vi "IV_.vi"(9 "B rate":dbl=0.02, 10 "Notes":string="LAOSTO110_2.K.20140812\n\nVbg=0.3V\nsweep Bx: 0T --> 1T --> -1T --> 0T, 0.02T/min\n\nLockin\n0:2\n1: 20\n2: 21\n3: 22\n4: 23\n5: 24\n\n", 11 "Experiment folder name":string="1 - sweep B,IV") -> ()   [LabVIEW 2013]
uses:
  <vilib>/Analysis/2dsp.llb/Decimate (single shot, DBL).vi
  <userlib>/LevyLab/PPMS VI/SubVI/ITX_Global.vi
  P:/users1/Joe/Lockin-4461_3.0 4461-4462 Multichannel Folder/DAQ-Lockin-SubVI/Lock-in Globles Multiple Inputs and Outputs.vi
  Q:/inst/Leiden measurements VIs/IV measurement/Sub VIs/Global Value.vi
  B field global.vi
  <vilib>/Analysis/NI_AALPro.lvlib
panel:
  out "4Term 2":cluster{dbl[], dbl[]}[](graph)
  out "4Term":cluster{dbl[], dbl[]}[](graph)
  out "2Term":cluster{dbl[], dbl[]}[](graph)
  in  "Tab Control":enum32{"Settings", "ITX", "Lockin Data"}(tab)
  in  "Current Channel 1":i32
  in  "Source Channel":i32
  in  "decimating factor":i32=400
  in  "low cutoff freq: fl":dbl=0.03 format="%0.4f"
  out "Gains":dbl[](array[numeric])=[50000000.0, 1000.0, 1000.0, 1000.0, 50000000.0, 1000.0]
  out "time":dbl[](array[numeric])=[3490742841.6947465, 3490742841.6967463, 3490742841.6987467, 3490742841.7007465, 3490742841.7027464, 3490742841.7047467, 3490742841.7067466, 3490742841.7087464, 3490742841.7107463, 3490742841.7127466, 3490742841.7147465, 3490742841.7167463, 3490742841.7187467, 3490742841.7207465, 3490742841.7227464, 3490742841.7247467, 3490742841.7267466, 3490742841.7287464, 3490742841.7307463, 3490742841.7327466, 3490742841.7347465, 3490742841.7367463, 3490742841.7387466, 3490742841.7407465, 3490742841.7427464, 3490742841.7447467, 3490742841.7467465, 3490742841.7487464, 3490742841.7507467, 3490742841.7527466, 3490742841.7547464, 3490742841.7567463, 3490742841.7587466, 3490742841.7607465, 3490742841.7627463, 3490742841.7647467, 3490742841.7667465, 3490742841.7687464, 3490742841.7707467, 3490742841.7727466, 3490742841.7747464, 3490742841.7767463, 3490742841.7787466, 3490742841.7807465, 3490742841.7827463, 3490742841.7847466, 3490742841.7867465, 3490742841.7887464, 3490742841.7907467, 3490742841.7927465, 3490742841.7947464, 3490742841.7967467, 3490742841.7987466, 3490742841.8007464, 3490742841.8027463, 3490742841.8047466, 3490742841.8067465, 3490742841.8087463, 3490742841.8107467, 3490742841.8127465, 3490742841.8147464, 3490742841.8167467, 3490742841.8187466, 3490742841.8207464, 3490742841.8227463, 3490742841.8247466, 3490742841.8267465, 3490742841.8287463, 3490742841.8307467, 3490742841.8327465, 3490742841.8347464, 3490742841.8367467, 3490742841.8387465, 3490742841.8407464, 3490742841.8427463, 3490742841.8447466, 3490742841.8467464, 3490742841.8487463, 3490742841.8507466, 3490742841.8527465, 3490742841.8547463, 3490742841.8567467, 3490742841.8587465, 3490742841.8607464, 3490742841.8627467, 3490742841.8647466, 3490742841.8667464, 3490742841.8687463, 3490742841.8707466, 3490742841.8727465, 3490742841.8747463, 3490742841.8767467, 3490742841.8787465, 3490742841.8807464, 3490742841.8827467, 3490742841.8847466, 3490742841.8867464, 3490742841.8887463, 3490742841.8907466, 3490742841.8927464, 3490742841.8947463, 3490742841.8967466, 3490742841.8987465, 3490742841.9007463, 3490742841.9027467, 3490742841.9047465, 3490742841.9067464, 3490742841.9087467, 3490742841.9107466, 3490742841.9127464, 3490742841.9147463, 3490742841.9167466, 3490742841.9187465, 3490742841.9207463, 3490742841.9227467, 3490742841.9247465, 3490742841.9267464, 3490742841.9287467, 3490742841.9307466, 3490742841.9327464, 3490742841.9347463, 3490742841.9367466, 3490742841.9387465, 3490742841.9407463, 3490742841.9427466, 3490742841.9447465, 3490742841.9467463, 3490742841.9487467, 3490742841.9507465, 3490742841.9527464, 3490742841.9547467, 3490742841.9567466, 3490742841.9587464, 3490742841.9607463, 3490742841.9627466, 3490742841.9647465, 3490742841.9667463, 3490742841.9687467, 3490742841.9707465, 3490742841.9727464, 3490742841.9747467, 3490742841.9767466, 3490742841.9787464, 3490742841.9807463, 3490742841.9827466, 3490742841.9847465, 3490742841.9867463, 3490742841.9887466, 3490742841.9907465, 3490742841.9927464, 3490742841.9947467, 3490742841.9967465, 3490742841.9987464, 3490742842.0007467, 3490742842.0027466, 3490742842.0047464, 3490742842.0067463, 3490742842.0087466, 3490742842.0107465, 3490742842.0127463, 3490742842.0147467, 3490742842.0167465, 3490742842.0187464, 3490742842.0207467, 3490742842.0227466, 3490742842.0247464, 3490742842.0267463, 3490742842.0287466, 3490742842.0307465, 3490742842.0327463, 3490742842.0347466, 3490742842.0367465, 3490742842.0387464, 3490742842.0407467, 3490742842.0427465, 3490742842.0447464, 3490742842.0467467, 3490742842.0487466, 3490742842.0507464, 3490742842.0527463, 3490742842.0547466, 3490742842.0567465, 3490742842.0587463, 3490742842.0607467, 3490742842.0627465, 3490742842.0647464, 3490742842.0667467, 3490742842.0687466, 3490742842.0707464, 3490742842.0727463, 3490742842.0747466, 3490742842.0767465, 3490742842.0787463, 3490742842.0807467, 3490742842.0827465, 3490742842.0847464, 3490742842.0867467, 3490742842.0887465, 3490742842.0907464, 3490742842.0927463, 3490742842.0947466, 3490742842.0967464, 3490742842.0987463, 3490742842.1007466, 3490742842.1027465, 3490742842.1047463, 3490742842.1067467, 3490742842.1087465, 3490742842.1107464, 3490742842.1127467, 3490742842.1147466, 3490742842.1167464, 3490742842.1187463, 3490742842.1207466, 3490742842.1227465, 3490742842.1247463, 3490742842.1267467, 3490742842.1287465, 3490742842.1307464, 3490742842.1327467, 3490742842.1347466, 3490742842.1367464, 3490742842.1387463, 3490742842.1407466, 3490742842.1427464, 3490742842.1447463, 3490742842.1467466, 3490742842.1487465, 3490742842.1507463, 3490742842.1527467, 3490742842.1547465, 3490742842.1567464, 3490742842.1587467, 3490742842.1607466, 3490742842.1627464, 3490742842.1647463, 3490742842.1667466, 3490742842.1687465, 3490742842.1707463, 3490742842.1727467, 3490742842.1747465, 3490742842.1767464, 3490742842.1787467, 3490742842.1807466, 3490742842.1827464, 3490742842.1847463, 3490742842.1867466, 3490742842.1887465, 3490742842.1907463, 3490742842.1927466, 3490742842.1947465, 3490742842.1967463, 3490742842.1987467, 3490742842.2007465, 3490742842.2027464, 3490742842.2047467, 3490742842.2067466, 3490742842.2087464, 3490742842.2107463, 3490742842.2127466, 3490742842.2147465, 3490742842.2167463, 3490742842.2187467, 3490742842.2207465, 3490742842.2227464, 3490742842.2247467, 3490742842.2267466, 3490742842.2287464, 3490742842.2307463, 3490742842.2327466, 3490742842.2347465, 3490742842.2367463, 3490742842.2387466, 3490742842.2407465, 3490742842.2427464, 3490742842.2447467, 3490742842.2467465, 3490742842.2487464, 3490742842.2507467, 3490742842.2527466, 3490742842.2547464, 3490742842.2567463, 3490742842.2587466, 3490742842.2607465, 3490742842.2627463, 3490742842.2647467, 3490742842.2667465, 3490742842.2687464, 3490742842.2707467, 3490742842.2727466, 3490742842.2747464, 3490742842.2767463, 3490742842.2787466, 3490742842.2807465, 3490742842.2827463, 3490742842.2847466, 3490742842.2867465, 3490742842.2887464, 3490742842.2907467, 3490742842.2927465, 3490742842.2947464, 3490742842.2967467, 3490742842.2987466, 3490742842.3007464, 3490742842.3027463, 3490742842.3047466, 3490742842.3067465, 3490742842.3087463, 3490742842.3107467, 3490742842.3127465, 3490742842.3147464, 3490742842.3167467, 3490742842.3187466, 3490742842.3207464, 3490742842.3227463, 3490742842.3247466, 3490742842.3267465, 3490742842.3287463, 3490742842.3307467, 3490742842.3327465, 3490742842.3347464, 3490742842.3367467, 3490742842.3387465, 3490742842.3407464, 3490742842.3427463, 3490742842.3447466, 3490742842.3467464, 3490742842.3487463, 3490742842.3507466, 3490742842.3527465, 3490742842.3547463, 3490742842.3567467, 3490742842.3587465, 3490742842.3607464, 3490742842.3627467, 3490742842.3647466, 3490742842.3667464, 3490742842.3687463, 3490742842.3707466, 3490742842.3727465, 3490742842.3747463, 3490742842.3767467, 3490742842.3787465, 3490742842.3807464, 3490742842.3827467, 3490742842.3847466, 3490742842.3867464, 3490742842.3887463, 3490742842.3907466, 3490742842.3927464, 3490742842.3947463, 3490742842.3967466, 3490742842.3987465, 3490742842.4007463, 3490742842.4027467, 3490742842.4047465, 3490742842.4067464, 3490742842.4087467, 3490742842.4107466, 3490742842.4127464, 3490742842.4147463, 3490742842.4167466, 3490742842.4187465, 3490742842.4207463, 3490742842.4227467, 3490742842.4247465, 3490742842.4267464, 3490742842.4287467, 3490742842.4307466, 3490742842.4327464, 3490742842.4347463, 3490742842.4367466, 3490742842.4387465, 3490742842.4407463, 3490742842.4427466, 3490742842.4447465, 3490742842.4467463, 3490742842.4487467, 3490742842.4507465, 3490742842.4527464, 3490742842.4547467, 3490742842.4567466, 3490742842.4587464, 3490742842.4607463, 3490742842.4627466, 3490742842.4647465, 3490742842.4667463, 3490742842.4687467, 3490742842.4707465, 3490742842.4727464, 3490742842.4747467, 3490742842.4767466, 3490742842.4787464, 3490742842.4807463, 3490742842.4827466, 3490742842.4847465, 3490742842.4867463, 3490742842.4887466, 3490742842.4907465, 3490742842.4927464, 3490742842.4947467, 3490742842.4967465, 3490742842.4987464, 3490742842.5007467, 3490742842.5027466, 3490742842.5047464, 3490742842.5067463, 3490742842.5087466, 3490742842.5107465, 3490742842.5127463, 3490742842.5147467, 3490742842.5167465, 3490742842.5187464, 3490742842.5207467, 3490742842.5227466, 3490742842.5247464, 3490742842.5267463, 3490742842.5287466, 3490742842.5307465, 3490742842.5327463, 3490742842.5347466, 3490742842.5367465, 3490742842.5387464, 3490742842.5407467, 3490742842.5427465, 3490742842.5447464, 3490742842.5467467, 3490742842.5487466, 3490742842.5507464, 3490742842.5527463, 3490742842.5547466, 3490742842.5567465, 3490742842.5587463, 3490742842.5607467, 3490742842.5627465, 3490742842.5647464, 3490742842.5667467, 3490742842.5687466, 3490742842.5707464, 3490742842.5727463, 3490742842.5747466, 3490742842.5767465, 3490742842.5787463, 3490742842.5807467, 3490742842.5827465, 3490742842.5847464, 3490742842.5867467, 3490742842.5887465, 3490742842.5907464, 3490742842.5927463, 3490742842.5947466, 3490742842.5967464, 3490742842.5987463, 3490742842.6007466, 3490742842.6027465, 3490742842.6047463, 3490742842.6067467, 3490742842.6087465, 3490742842.6107464, 3490742842.6127467, 3490742842.6147466, 3490742842.6167464, 3490742842.6187463, 3490742842.6207466, 3490742842.6227465, 3490742842.6247463, 3490742842.6267467, 3490742842.6287465, 3490742842.6307464, 3490742842.6327467, 3490742842.6347466, 3490742842.6367464, 3490742842.6387463, 3490742842.6407466, 3490742842.6427464, 3490742842.6447463, 3490742842.6467466, 3490742842.6487465, 3490742842.6507463, 3490742842.6527467, 3490742842.6547465, 3490742842.6567464, 3490742842.6587467, 3490742842.6607466, 3490742842.6627464, 3490742842.6647463, 3490742842.6667466, 3490742842.6687465, 3490742842.6707463, 3490742842.6727467, 3490742842.6747465, 3490742842.6767464, 3490742842.6787467, 3490742842.6807466, 3490742842.6827464, 3490742842.6847463, 3490742842.6867466, 3490742842.6887465, 3490742842.6907463, 3490742842.6927466, 3490742842.6947465, 3490742842.6967463, 3490742842.6987467, 3490742842.7007465, 3490742842.7027464, 3490742842.7047467, 3490742842.7067466, 3490742842.7087464, 3490742842.7107463, 3490742842.7127466, 3490742842.7147465, 3490742842.7167463, 3490742842.7187467, 3490742842.7207465, 3490742842.7227464, 3490742842.7247467, 3490742842.7267466, 3490742842.7287464, 3490742842.7307463, 3490742842.7327466, 3490742842.7347465, 3490742842.7367463, 3490742842.7387466, 3490742842.7407465, 3490742842.7427464, 3490742842.7447467, 3490742842.7467465, 3490742842.7487464, 3490742842.7507467, 3490742842.7527466, 3490742842.7547464, 3490742842.7567463, 3490742842.7587466, 3490742842.7607465, 3490742842.7627463, 3490742842.7647467, 3490742842.7667465, 3490742842.7687464, 3490742842.7707467, 3490742842.7727466, 3490742842.7747464, 3490742842.7767463, 3490742842.7787466, 3490742842.7807465, 3490742842.7827463, 3490742842.7847466, 3490742842.7867465, 3490742842.7887464, 3490742842.7907467, 3490742842.7927465, 3490742842.7947464, 3490742842.7967467, 3490742842.7987466, 3490742842.8007464, 3490742842.8027463, 3490742842.8047466, 3490742842.8067465, 3490742842.8087463, 3490742842.8107467, 3490742842.8127465, 3490742842.8147464, 3490742842.8167467, 3490742842.8187466, 3490742842.8207464, 3490742842.8227463, 3490742842.8247466, 3490742842.8267465, 3490742842.8287463, 3490742842.8307467, 3490742842.8327465, 3490742842.8347464, 3490742842.8367467, 3490742842.8387465, 3490742842.8407464, 3490742842.8427463, 3490742842.8447466, 3490742842.8467464, 3490742842.8487463, 3490742842.8507466, 3490742842.8527465, 3490742842.8547463, 3490742842.8567467, 3490742842.8587465, 3490742842.8607464, 3490742842.8627467, 3490742842.8647466, 3490742842.8667464, 3490742842.8687463, 3490742842.8707466, 3490742842.8727465, 3490742842.8747463, 3490742842.8767467, 3490742842.8787465, 3490742842.8807464, 3490742842.8827467, 3490742842.8847466, 3490742842.8867464, 3490742842.8887463, 3490742842.8907466, 3490742842.8927464, 3490742842.8947463, 3490742842.8967466, 3490742842.8987465, 3490742842.9007463, 3490742842.9027467, 3490742842.9047465, 3490742842.9067464, 3490742842.9087467, 3490742842.9107466, 3490742842.9127464, 3490742842.9147463, 3490742842.9167466, 3490742842.9187465, 3490742842.9207463, 3490742842.9227467, 3490742842.9247465, 3490742842.9267464, 3490742842.9287467, 3490742842.9307466, 3490742842.9327464, 3490742842.9347463, 3490742842.9367466, 3490742842.9387465, 3490742842.9407463, 3490742842.9427466, 3490742842.9447465, 3490742842.9467463, 3490742842.9487467, 3490742842.9507465, 3490742842.9527464, 3490742842.9547467, 3490742842.9567466, 3490742842.9587464, 3490742842.9607463, 3490742842.9627466, 3490742842.9647465, 3490742842.9667463, 3490742842.9687467, 3490742842.9707465, 3490742842.9727464, 3490742842.9747467, 3490742842.9767466, 3490742842.9787464, 3490742842.9807463, 3490742842.9827466, 3490742842.9847465, 3490742842.9867463, 3490742842.9887466, 3490742842.9907465, 3490742842.9927464, 3490742842.9947467, 3490742842.9967465, 3490742842.9987464, 3490742843.0007467, 3490742843.0027466, 3490742843.0047464, 3490742843.0067463, 3490742843.0087466, 3490742843.0107465, 3490742843.0127463, 3490742843.0147467, 3490742843.0167465, 3490742843.0187464, 3490742843.0207467, 3490742843.0227466, 3490742843.0247464, 3490742843.0267463, 3490742843.0287466, 3490742843.0307465, 3490742843.0327463, 3490742843.0347466, 3490742843.0367465, 3490742843.0387464, 3490742843.0407467, 3490742843.0427465, 3490742843.0447464, 3490742843.0467467, 3490742843.0487466, 3490742843.0507464, 3490742843.0527463, 3490742843.0547466, 3490742843.0567465, 3490742843.0587463, 3490742843.0607467, 3490742843.0627465, 3490742843.0647464, 3490742843.0667467, 3490742843.0687466, 3490742843.0707464, 3490742843.0727463, 3490742843.0747466, 3490742843.0767465, 3490742843.0787463, 3490742843.0807467, 3490742843.0827465, 3490742843.0847464, 3490742843.0867467, 3490742843.0887465, 3490742843.0907464, 3490742843.0927463, 3490742843.0947466, 3490742843.0967464, 3490742843.0987463, 3490742843.1007466, 3490742843.1027465, 3490742843.1047463, 3490742843.1067467, 3490742843.1087465, 3490742843.1107464, 3490742843.1127467, 3490742843.1147466, 3490742843.1167464, 3490742843.1187463, 3490742843.1207466, 3490742843.1227465, 3490742843.1247463, 3490742843.1267467, 3490742843.1287465, 3490742843.1307464, 3490742843.1327467, 3490742843.1347466, 3490742843.1367464, 3490742843.1387463, 3490742843.1407466, 3490742843.1427464, 3490742843.1447463, 3490742843.1467466, 3490742843.1487465, 3490742843.1507463, 3490742843.1527467, 3490742843.1547465, 3490742843.1567464, 3490742843.1587467, 3490742843.1607466, 3490742843.1627464, 3490742843.1647463, 3490742843.1667466, 3490742843.1687465, 3490742843.1707463, 3490742843.1727467, 3490742843.1747465, 3490742843.1767464, 3490742843.1787467, 3490742843.1807466, 3490742843.1827464, 3490742843.1847463, 3490742843.1867466, 3490742843.1887465, 3490742843.1907463, 3490742843.1927466, 3490742843.1947465, 3490742843.1967463, 3490742843.1987467, 3490742843.2007465, 3490742843.2027464, 3490742843.2047467, 3490742843.2067466, 3490742843.2087464, 3490742843.2107463, 3490742843.2127466, 3490742843.2147465, 3490742843.2167463, 3490742843.2187467, 3490742843.2207465, 3490742843.2227464, 3490742843.2247467, 3490742843.2267466, 3490742843.2287464, 3490742843.2307463, 3490742843.2327466, 3490742843.2347465, 3490742843.2367463, 3490742843.2387466, 3490742843.2407465, 3490742843.2427464, 3490742843.2447467, 3490742843.2467465, 3490742843.2487464, 3490742843.2507467, 3490742843.2527466, 3490742843.2547464, 3490742843.2567463, 3490742843.2587466, 3490742843.2607465, 3490742843.2627463, 3490742843.2647467, 3490742843.2667465, 3490742843.2687464, 3490742843.2707467, 3490742843.2727466, 3490742843.2747464, 3490742843.2767463, 3490742843.2787466, 3490742843.2807465, 3490742843.2827463, 3490742843.2847466, 3490742843.2867465, 3490742843.2887464, 3490742843.2907467, 3490742843.2927465, 3490742843.2947464, 3490742843.2967467, 3490742843.2987466, 3490742843.3007464, 3490742843.3027463, 3490742843.3047466, 3490742843.3067465, 3490742843.3087463, 3490742843.3107467, 3490742843.3127465, 3490742843.3147464, 3490742843.3167467, 3490742843.3187466, 3490742843.3207464, 3490742843.3227463, 3490742843.3247466, 3490742843.3267465, 3490742843.3287463, 3490742843.3307467, 3490742843.3327465, 3490742843.3347464, 3490742843.3367467, 3490742843.3387465, 3490742843.3407464, 3490742843.3427463, 3490742843.3447466, 3490742843.3467464, 3490742843.3487463, 3490742843.3507466, 3490742843.3527465, 3490742843.3547463, 3490742843.3567467, 3490742843.3587465, 3490742843.3607464, 3490742843.3627467, 3490742843.3647466, 3490742843.3667464, 3490742843.3687463, 3490742843.3707466, 3490742843.3727465, 3490742843.3747463, 3490742843.3767467, 3490742843.3787465, 3490742843.3807464, 3490742843.3827467, 3490742843.3847466, 3490742843.3867464, 3490742843.3887463, 3490742843.3907466, 3490742843.3927464, 3490742843.3947463, 3490742843.3967466, 3490742843.3987465, 3490742843.4007463, 3490742843.4027467, 3490742843.4047465, 3490742843.4067464, 3490742843.4087467, 3490742843.4107466, 3490742843.4127464, 3490742843.4147463, 3490742843.4167466, 3490742843.4187465, 3490742843.4207463, 3490742843.4227467, 3490742843.4247465, 3490742843.4267464, 3490742843.4287467, 3490742843.4307466, 3490742843.4327464, 3490742843.4347463, 3490742843.4367466, 3490742843.4387465, 3490742843.4407463, 3490742843.4427466, 3490742843.4447465, 3490742843.4467463, 3490742843.4487467, 3490742843.4507465, 3490742843.4527464, 3490742843.4547467, 3490742843.4567466, 3490742843.4587464, 3490742843.4607463, 3490742843.4627466, 3490742843.4647465, 3490742843.4667463, 3490742843.4687467, 3490742843.4707465, 3490742843.4727464, 3490742843.4747467, 3490742843.4767466, 3490742843.4787464, 3490742843.4807463, 3490742843.4827466, 3490742843.4847465, 3490742843.4867463, 3490742843.4887466, 3490742843.4907465, 3490742843.4927464, 3490742843.4947467, 3490742843.4967465, 3490742843.4987464, 3490742843.5007467, 3490742843.5027466, 3490742843.5047464, 3490742843.5067463, 3490742843.5087466, 3490742843.5107465, 3490742843.5127463, 3490742843.5147467, 3490742843.5167465, 3490742843.5187464, 3490742843.5207467, 3490742843.5227466, 3490742843.5247464, 3490742843.5267463, 3490742843.5287466, 3490742843.5307465, 3490742843.5327463, 3490742843.5347466, 3490742843.5367465, 3490742843.5387464, 3490742843.5407467, 3490742843.5427465, 3490742843.5447464, 3490742843.5467467, 3490742843.5487466, 3490742843.5507464, 3490742843.5527463, 3490742843.5547466, 3490742843.5567465, 3490742843.5587463, 3490742843.5607467, 3490742843.5627465, 3490742843.5647464, 3490742843.5667467, 3490742843.5687466, 3490742843.5707464, 3490742843.5727463, 3490742843.5747466, 3490742843.5767465, 3490742843.5787463, 3490742843.5807467, 3490742843.5827465, 3490742843.5847464, 3490742843.5867467, 3490742843.5887465, 3490742843.5907464, 3490742843.5927463, 3490742843.5947466, 3490742843.5967464, 3490742843.5987463, 3490742843.6007466, 3490742843.6027465, 3490742843.6047463, 3490742843.6067467, 3490742843.6087465, 3490742843.6107464, 3490742843.6127467, 3490742843.6147466, 3490742843.6167464, 3490742843.6187463, 3490742843.6207466, 3490742843.6227465, 3490742843.6247463, 3490742843.6267467, 3490742843.6287465, 3490742843.6307464, 3490742843.6327467, 3490742843.6347466, 3490742843.6367464, 3490742843.6387463, 3490742843.6407466, 3490742843.6427464, 3490742843.6447463, 3490742843.6467466, 3490742843.6487465, 3490742843.6507463, 3490742843.6527467, 3490742843.6547465, 3490742843.6567464, 3490742843.6587467, 3490742843.6607466, 3490742843.6627464, 3490742843.6647463, 3490742843.6667466, 3490742843.6687465, 3490742843.6707463, 3490742843.6727467, 3490742843.6747465, 3490742843.6767464, 3490742843.6787467, 3490742843.6807466, 3490742843.6827464, 3490742843.6847463, 3490742843.6867466, 3490742843.6887465, 3490742843.6907463, 3490742843.6927466, 3490742843.6947465, 3490742843.6967463, 3490742843.6987467, 3490742843.7007465, 3490742843.7027464, 3490742843.7047467, 3490742843.7067466, 3490742843.7087464, 3490742843.7107463, 3490742843.7127466, 3490742843.7147465, 3490742843.7167463, 3490742843.7187467, 3490742843.7207465, 3490742843.7227464, 3490742843.7247467, 3490742843.7267466, 3490742843.7287464, 3490742843.7307463, 3490742843.7327466, 3490742843.7347465, 3490742843.7367463, 3490742843.7387466, 3490742843.7407465, 3490742843.7427464, 3490742843.7447467, 3490742843.7467465, 3490742843.7487464, 3490742843.7507467, 3490742843.7527466, 3490742843.7547464, 3490742843.7567463, 3490742843.7587466, 3490742843.7607465, 3490742843.7627463, 3490742843.7647467, 3490742843.7667465, 3490742843.7687464, 3490742843.7707467, 3490742843.7727466, 3490742843.7747464, 3490742843.7767463, 3490742843.7787466, 3490742843.7807465, 3490742843.7827463, 3490742843.7847466, 3490742843.7867465, 3490742843.7887464, 3490742843.7907467, 3490742843.7927465, 3490742843.7947464, 3490742843.7967467, 3490742843.7987466, 3490742843.8007464, 3490742843.8027463, 3490742843.8047466, 3490742843.8067465, 3490742843.8087463, 3490742843.8107467, 3490742843.8127465, 3490742843.8147464, 3490742843.8167467, 3490742843.8187466, 3490742843.8207464, 3490742843.8227463, 3490742843.8247466, 3490742843.8267465, 3490742843.8287463, 3490742843.8307467, 3490742843.8327465, 3490742843.8347464, 3490742843.8367467, 3490742843.8387465, 3490742843.8407464, 3490742843.8427463, 3490742843.8447466, 3490742843.8467464, 3490742843.8487463, 3490742843.8507466, 3490742843.8527465, 3490742843.8547463, 3490742843.8567467, 3490742843.8587465, 3490742843.8607464, 3490742843.8627467, 3490742843.8647466, 3490742843.8667464, 3490742843.8687463, 3490742843.8707466, 3490742843.8727465, 3490742843.8747463, 3490742843.8767467, 3490742843.8787465, 3490742843.8807464, 3490742843.8827467, 3490742843.8847466, 3490742843.8867464, 3490742843.8887463, 3490742843.8907466, 3490742843.8927464, 3490742843.8947463, 3490742843.8967466, 3490742843.8987465, 3490742843.9007463, 3490742843.9027467, 3490742843.9047465, 3490742843.9067464, 3490742843.9087467, 3490742843.9107466, 3490742843.9127464, 3490742843.9147463, 3490742843.9167466, 3490742843.9187465, 3490742843.9207463, 3490742843.9227467, 3490742843.9247465, 3490742843.9267464, 3490742843.9287467, 3490742843.9307466, 3490742843.9327464, 3490742843.9347463, 3490742843.9367466, 3490742843.9387465, 3490742843.9407463, 3490742843.9427466, 3490742843.9447465, 3490742843.9467463, 3490742843.9487467, 3490742843.9507465, 3490742843.9527464, 3490742843.9547467, 3490742843.9567466, 3490742843.9587464, 3490742843.9607463, 3490742843.9627466, 3490742843.9647465, 3490742843.9667463, 3490742843.9687467, 3490742843.9707465, 3490742843.9727464, 3490742843.9747467, 3490742843.9767466, 3490742843.9787464, 3490742843.9807463, 3490742843.9827466, 3490742843.9847465, 3490742843.9867463, 3490742843.9887466, 3490742843.9907465, 3490742843.9927464, 3490742843.9947467, 3490742843.9967465, 3490742843.9987464, 3490742844.0007467, 3490742844.0027466, 3490742844.0047464, 3490742844.0067463, 3490742844.0087466, 3490742844.0107465, 3490742844.0127463, 3490742844.0147467, 3490742844.0167465, 3490742844.0187464, 3490742844.0207467, 3490742844.0227466, 3490742844.0247464, 3490742844.0267463, 3490742844.0287466, 3490742844.0307465, 3490742844.0327463, 3490742844.0347466, 3490742844.0367465, 3490742844.0387464, 3490742844.0407467, 3490742844.0427465, 3490742844.0447464, 3490742844.0467467, 3490742844.0487466, 3490742844.0507464, 3490742844.0527463, 3490742844.0547466, 3490742844.0567465, 3490742844.0587463, 3490742844.0607467, 3490742844.0627465, 3490742844.0647464, 3490742844.0667467, 3490742844.0687466, 3490742844.0707464, 3490742844.0727463, 3490742844.0747466, 3490742844.0767465, 3490742844.0787463, 3490742844.0807467, 3490742844.0827465, 3490742844.0847464, 3490742844.0867467, 3490742844.0887465, 3490742844.0907464, 3490742844.0927463, 3490742844.0947466, 3490742844.0967464, 3490742844.0987463, 3490742844.1007466, 3490742844.1027465, 3490742844.1047463, 3490742844.1067467, 3490742844.1087465, 3490742844.1107464, 3490742844.1127467, 3490742844.1147466, 3490742844.1167464, 3490742844.1187463, 3490742844.1207466, 3490742844.1227465, 3490742844.1247463, 3490742844.1267467, 3490742844.1287465, 3490742844.1307464, 3490742844.1327467, 3490742844.1347466, 3490742844.1367464, 3490742844.1387463, 3490742844.1407466, 3490742844.1427464, 3490742844.1447463, 3490742844.1467466, 3490742844.1487465, 3490742844.1507463, 3490742844.1527467, 3490742844.1547465, 3490742844.1567464, 3490742844.1587467, 3490742844.1607466, 3490742844.1627464, 3490742844.1647463, 3490742844.1667466, 3490742844.1687465, 3490742844.1707463, 3490742844.1727467, 3490742844.1747465, 3490742844.1767464, 3490742844.1787467, 3490742844.1807466, 3490742844.1827464, 3490742844.1847463, 3490742844.1867466, 3490742844.1887465, 3490742844.1907463, 3490742844.1927466]
  out "Temp":dbl=34.357534
  out "B fields":dbl[](array[numeric])
  in  "wait":u32=5000
  in  "Current Channel 2":i32=4
  in  "offset":dbl[](array[numeric])=[0.0, -3e-10, 0.0, 4e-05, 0.0, -8e-10] format="%_6p"
  in  "invert":dbl[](array[numeric])=[-1.0, 1.0, 1.0, 1.0, 1.0, 1.0] format="%#_6p"
  out "DC Voltages":dbl[](array[numeric])
  in  "save?":bool=TRUE
  out "Input signal":dbl[][](graph)
  out "output":dbl[][](graph)
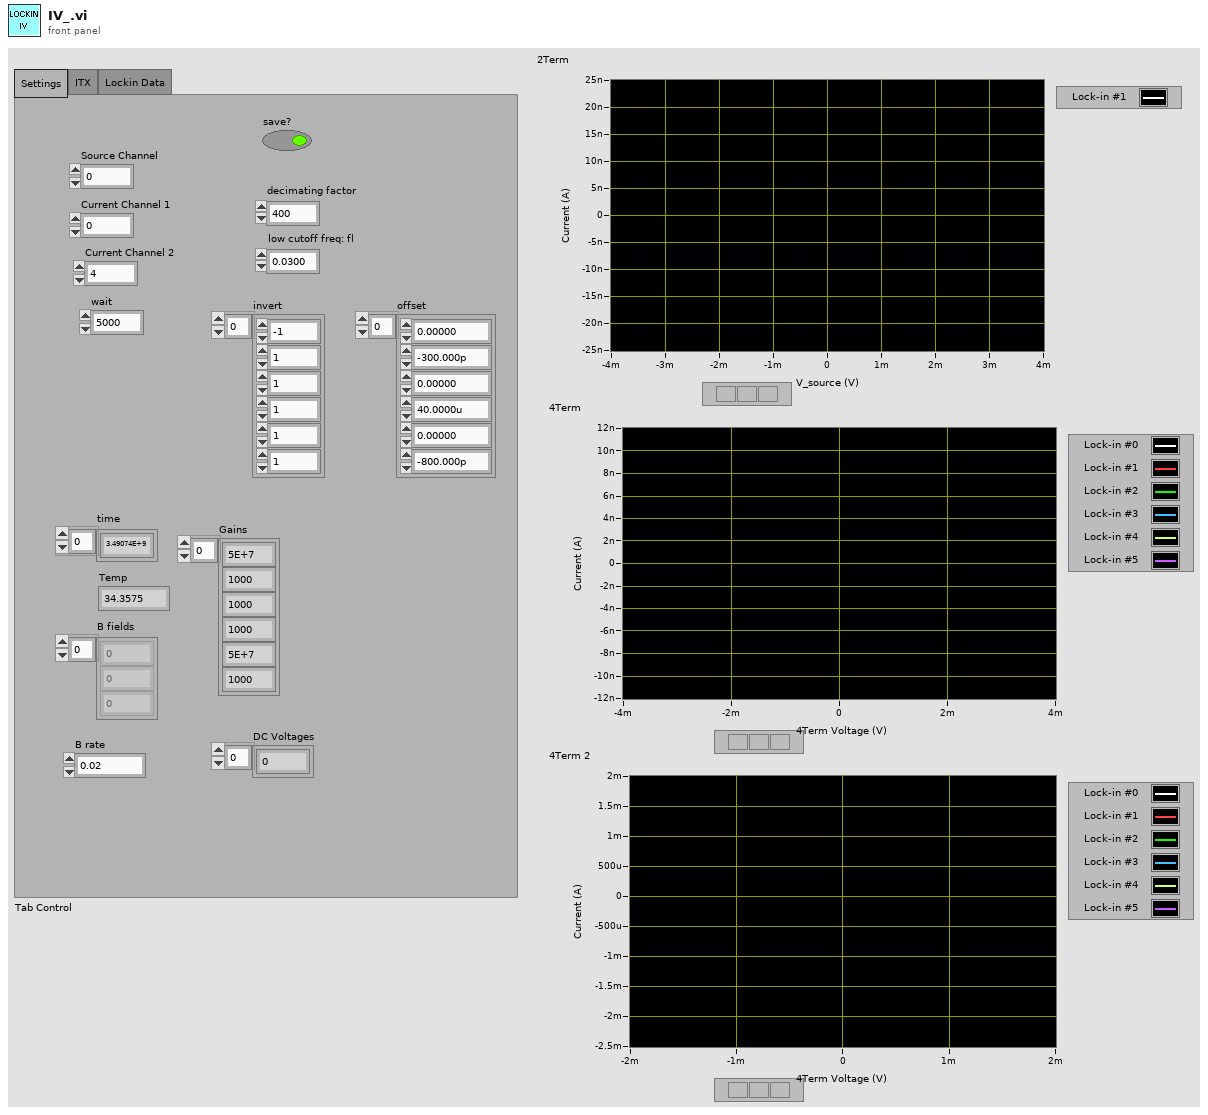
[diagram p1: front panel]
types:
  T1 = cluster{"Signal Type":enum16{"Sine Wave", "Triangle Wave", "Square Wave", "Sawtooth Wave"}, "DC":dbl, "Amplitude":dbl, "frequency":dbl, "Phase":dbl}[][]
  T2 = cluster{"Channel":u16, "Gain":u16, "Shunt Resistor":u16, "Measure":u16}[]
  T3 = cluster{"Decimated Array":dbl[], "Decimated Array":dbl[]}
  T4 = cluster{"Decimated Array":dbl[], "Decimated Array":dbl[]}[]
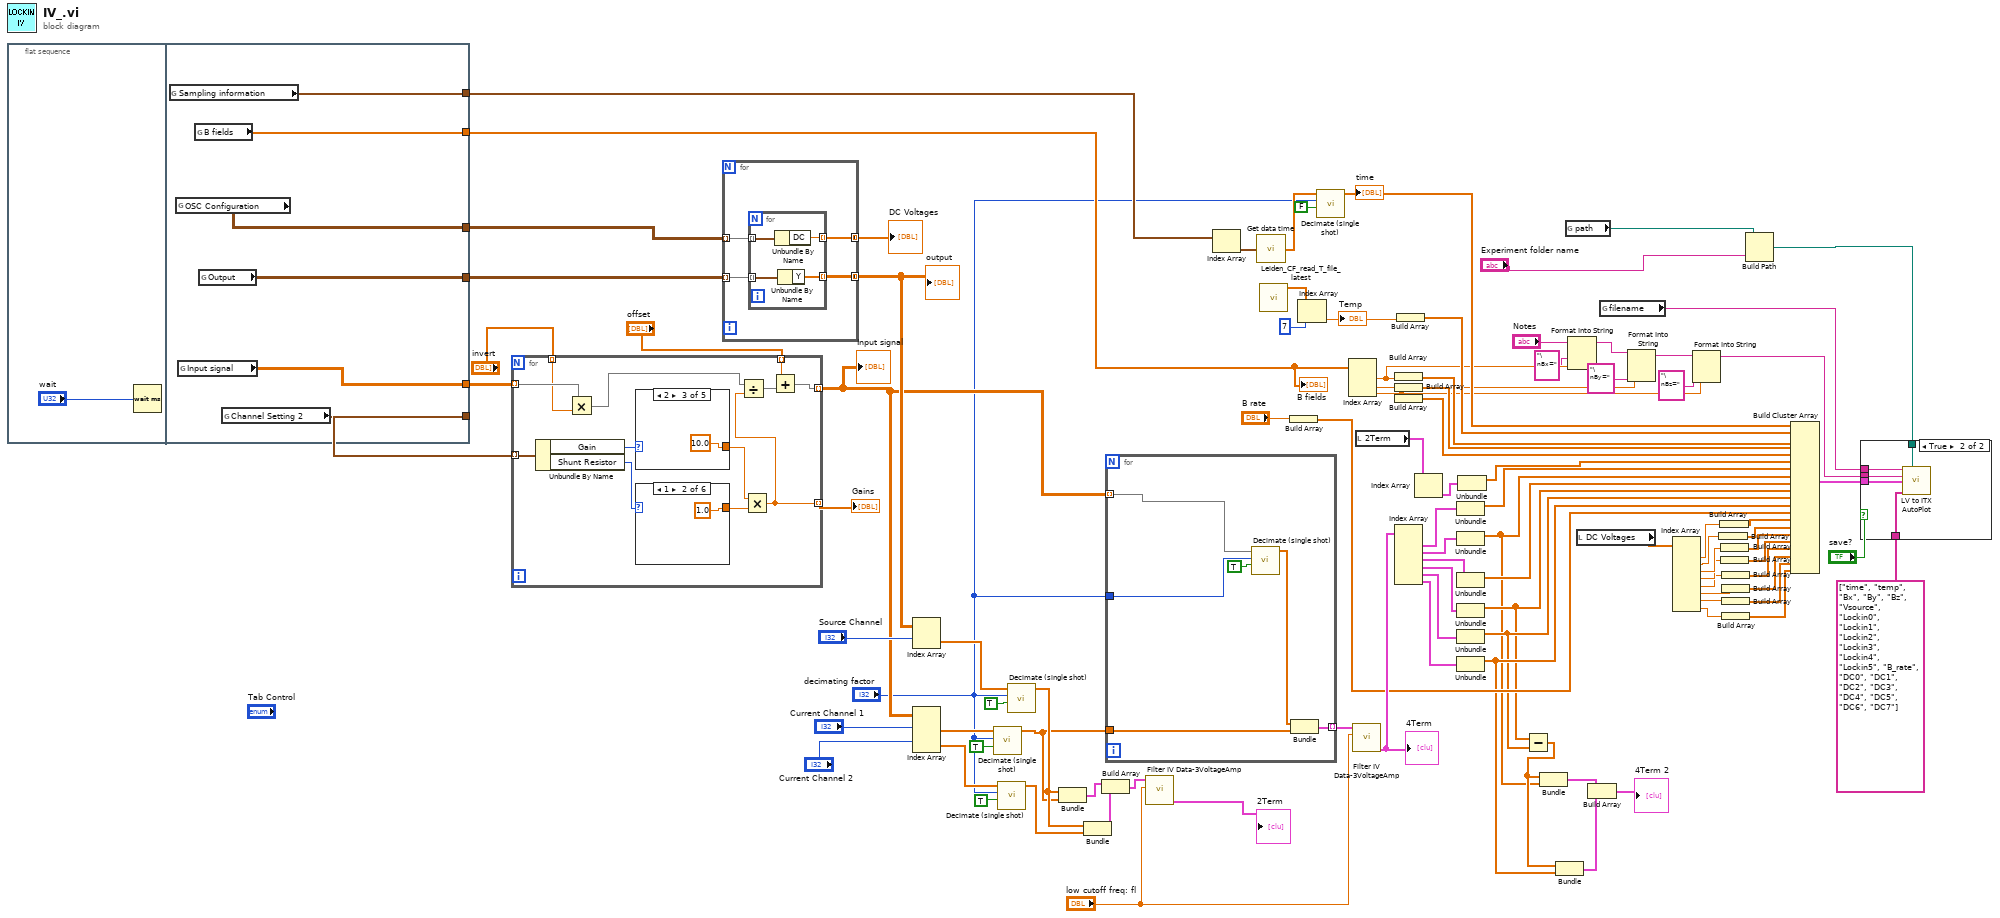
[diagram p0: block diagram]
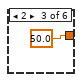
[diagram p4: hidden frame]
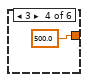
[diagram p5: hidden frame]
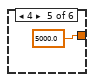
[diagram p6: hidden frame]
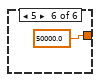
[diagram p7: hidden frame]
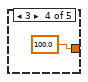
[diagram p10: hidden frame]
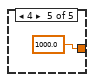
[diagram p11: hidden frame]
diagram:
  n1 = flat-sequence {
    tunnel: [w105] -> w98
    tunnel: [w100] -> w30
    tunnel: [w104] -> w29
    tunnel: [w103] -> w28
    tunnel: [w102] -> w27
    tunnel: [w101] -> w26
    frame #0 {
      n2 = Wait (ms)(milliseconds to wait="wait") -> ()  [unwired: 1 out]
    }
    frame #1 {
      n3 = global read "Lock-in Globles Multiple Inputs and Outputs.vi" "Sampling information"() -> (w102:cluster{"Fs":dbl, "#s":dbl}[])
      n4 = global read "Lock-in Globles Multiple Inputs and Outputs.vi" "OSC Configuration"() -> (w100:T1)
      n5 = global read "Lock-in Globles Multiple Inputs and Outputs.vi" "Input signal"() -> (w105:dbl[][])
      n6 = global read "B field global.vi" "B fields"() -> (w101:dbl[])
      n7 = global read "Lock-in Globles Multiple Inputs and Outputs.vi" "Output"() -> (w104:waveform(dbl)[][])
      n8 = global read "Global Value.vi" "Channel Setting 2"() -> (w103:T2)
    }
  }
  n9 = for {
    tunnel: w28 -> [w115] mode=indexing
    tunnel: [w112] -> w97 mode=indexing
    tunnel: w98 -> [w108] mode=indexing
    tunnel: [w110] -> w53 mode=indexing
    tunnel: "offset" -> [w109] mode=indexing
    tunnel: "invert" -> [w107] mode=indexing
    n10 = Unbundle By Name(w115) -> ("Gain"=w114:u16, "Shunt Resistor"=w113:u16)
    n11 = Multiply(x=w108, y=w107) -> (x*y=w106:dbl[])
    n12 = case shown="2" w114 {
      selector: w114 -> [w124 w125 _ _ _]
      tunnel: [w124 w125 10.0 100.0 1000.0] -> w117
      frame 0, Default {
      }
      frame 1 {
      }
      frame 2 {
      }
      frame 3 {
      }
      frame 4 {
      }
    }
    n13 = case shown="1" w113 {
      selector: w113 -> [w118 _ _ _ _ _]
      tunnel: [w118 1.0 50.0 500.0 5000.0 50000.0] -> w116
      frame 0, Default {
      }
      frame 1 {
      }
      frame 2 {
      }
      frame 3 {
      }
      frame 4 {
      }
      frame 5 {
      }
    }
    n14 = Multiply(x=w117, y=w116) -> (x*y=w112:dbl)
    n15 = Divide(x=w106, y=w112) -> (x/y=w111:dbl[])
    n16 = Add(x=w109, y=w111) -> (x+y=w110:dbl[])
  }
  "Input signal" <- w53
  "Gains" <- w97
  n17 = for {
    tunnel: w29 -> [w132] mode=indexing
    tunnel: [w131] -> w91 mode=concatenating
    tunnel: w30 -> [w130] mode=indexing
    tunnel: [w129] -> w48 mode=concatenating
    n18 = for {
      tunnel: w132 -> [w136] mode=indexing
      tunnel: [w135] -> w131 mode=indexing
      tunnel: w130 -> [w134] mode=indexing
      tunnel: [w133] -> w129 mode=indexing
      n19 = Unbundle By Name(w134) -> ("DC"=w133:dbl)
      n20 = Unbundle By Name(w136) -> ("Y"=w135:dbl[])
    }
  }
  "output" <- w91
  "DC Voltages" <- w48
  n21 = Index Array(array=w91, index (row)="Source Channel") -> (element=w72:dbl[])  [unwired: 1 in]
  n22 = Index Array(array=w53, index (row) #1="Current Channel 1", index (row) #2="Current Channel 2") -> (element #1=w16:dbl[], element #2=w15:dbl[])  [unwired: 2 in]
  n23 = call-poly <vilib>:"Decimate (single shot).vi"("averaging"=TRUE, "decimating factor"="decimating factor", "X"=w16) -> ("Decimated Array"=w23:dbl[])  [unwired: 7 in, 1 out]
  n24 = call-poly <vilib>:"Decimate (single shot).vi"("averaging"=TRUE, "decimating factor"="decimating factor", "X"=w15) -> ("Decimated Array"=w22:dbl[])  [unwired: 7 in, 1 out]
  n25 = call-poly <vilib>:"Decimate (single shot).vi"("averaging"=TRUE, "decimating factor"="decimating factor", "X"=w72) -> ("Decimated Array"=w24:dbl[])  [unwired: 7 in, 1 out]
  n26 = Bundle("Decimated Array"=w24, "Decimated Array"=w23) -> (w25:T3)  [unwired: 1 in]
  n27 = Bundle("Decimated Array"=w24, "Decimated Array"=w22) -> (w21:T3)  [unwired: 1 in]
  n28 = Build Array(w25, w21) -> (w17:T4)
  n29 = for {
    tunnel: w53 -> [w137] mode=indexing
    tunnel: "decimating factor" -> [w141]
    tunnel: w23 -> [w140]
    tunnel: [w138] -> w71 mode=indexing
    n30 = call-poly <vilib>:"Decimate (single shot).vi"("averaging"=TRUE, "decimating factor"=w141, "X"=w137) -> ("Decimated Array"=w139:dbl[])  [unwired: 7 in, 1 out]
    n31 = Bundle("Decimated Array"=w139, "Decimated Array"=w140) -> (w138:T3)  [unwired: 1 in]
  }
  n32 = call <userlib>:"Filter IV Data-3VoltageAmp.vi"("low cutoff freq: fl"="low cutoff freq: fl", "IVs"=w17) -> ("V vs I 2"=→"2Term":cluster{dbl[], dbl[]}[])  [unwired: 1 in]
  n33 = Index Array(array=w27) -> (element=w90:cluster{"Fs":dbl, "#s":dbl})  [unwired: 1 in]
  n34 = call <userlib>:"Get data time.vi"("sampling info"=w90) -> ("Array"=w88:dbl[])
  n35 = call "Leiden_CF_read_T_file_latest.vi"() -> ("T array"=w87:dbl[])  [unwired: 11 in]
  n36 = Build Array("B rate") -> (w60:dbl[])
  n37 = Index Array(array=w87, index=7) -> (element=w79:dbl)
  "Temp" <- w79
  n38 = call-poly <vilib>:"Decimate (single shot).vi"("averaging"=FALSE, "decimating factor"="decimating factor", "X"=w88) -> ("Decimated Array"=w80:dbl[])  [unwired: 7 in, 1 out]
  "time" <- w80
  n39 = Index Array(array=w26) -> (element #1=w10:dbl, element #2=w8:dbl, element #3=w7:dbl)  [unwired: 3 in]
  n40 = call <userlib>:"Filter IV Data-3VoltageAmp.vi"("low cutoff freq: fl"="low cutoff freq: fl", "IVs"=w71) -> ("V vs I 2"=w70:cluster{dbl[], dbl[]}[])  [unwired: 1 in]
  "4Term" <- w70
  n41 = local read "2Term"() -> (w19:cluster{dbl[], dbl[]}[])
  n42 = Build Array(w10) -> (w77:dbl[])
  n43 = Build Array(w8) -> (w76:dbl[])
  n44 = Build Array(w7) -> (w75:dbl[])
  n45 = Index Array(array=w70) -> (element #1=w69:cluster{dbl[], dbl[]}, element #2=w68:cluster{dbl[], dbl[]}, element #3=w67:cluster{dbl[], dbl[]}, element #4=w66:cluster{dbl[], dbl[]}, element #5=w65:cluster{dbl[], dbl[]}, element #6=w64:cluster{dbl[], dbl[]})  [unwired: 6 in]
  n46 = Build Array(w79) -> (w78:dbl[])
  n47 = Index Array(array=w19) -> (element=w18:cluster{dbl[], dbl[]})  [unwired: 1 in]
  n48 = Unbundle(w69) -> (w63:dbl[])  [unwired: 1 out]
  n49 = Unbundle(w68) -> (w12:dbl[])  [unwired: 1 out]
  n50 = Unbundle(w67) -> (w62:dbl[])  [unwired: 1 out]
  n51 = Unbundle(w66) -> (w57:dbl[])  [unwired: 1 out]
  n52 = Unbundle(w65) -> (w58:dbl[])  [unwired: 1 out]
  n53 = Unbundle(w64) -> (w59:dbl[])  [unwired: 1 out]
  n54 = Unbundle(w18) -> (w73:dbl[])  [unwired: 1 out]
  n55 = Subtract(x=w57, y=w58) -> (x-y=w13:dbl[])
  n56 = Bundle(w13, w12) -> (w55:cluster{dbl[], dbl[]})  [unwired: 1 in]
  n57 = Bundle(w13, w59) -> (w56:cluster{dbl[], dbl[]})  [unwired: 1 in]
  n58 = global read "ITX_Global.vi" "path"() -> (w85:path)
  n59 = Format Into String(initial string="Notes", "\nBx=" ("input 1"), w10) -> (resulting string=w4:string)  [unwired: 2 in, 1 out]
  n60 = local read "DC Voltages"() -> (w47:dbl[])
  n61 = Build Array(w55, w56) -> (→"4Term 2":cluster{dbl[], dbl[]}[])
  n62 = global read "ITX_Global.vi" "filename"() -> (w82:string)
  n63 = Format Into String(initial string=w4, "\nBy=" ("input 1"), w8) -> (resulting string=w3:string)  [unwired: 2 in, 1 out]
  n64 = Index Array(array=w47) -> (element #1=w46:dbl, element #2=w44:dbl, element #3=w42:dbl, element #4=w40:dbl, element #5=w38:dbl, element #6=w36:dbl, element #7=w34:dbl, element #8=w32:dbl)  [unwired: 8 in]
  n65 = Format Into String(initial string=w3, "\nBz=" ("input 1"), w7) -> (resulting string=w9:string)  [unwired: 2 in, 1 out]
  n66 = Build Array(w44) -> (w43:dbl[])
  n67 = Build Array(w46) -> (w45:dbl[])
  n68 = Build Array(w42) -> (w41:dbl[])
  n69 = Build Array(w40) -> (w39:dbl[])
  n70 = Build Array(w38) -> (w37:dbl[])
  n71 = Build Array(w36) -> (w35:dbl[])
  n72 = Build Array(w34) -> (w33:dbl[])
  n73 = Build Array(w32) -> (w31:dbl[])
  n74 = Build Path(base path=w85, name or relative path="Experiment folder name") -> (appended path=w83:path)
  n75 = Build Cluster Array(w80, w78, w77, w76, w75, w73, w63, w12, w62, w57, w58, w59, w60, w45, w43, w41, w39, w37, w35, w33, w31) -> (w74:cluster{"Decimated Array":dbl[]}[])
  n76 = case shown="True" "save?" {
    tunnel: w83 -> [_ w147]
    tunnel: w9 -> [_ w146]
    tunnel: w82 -> [_ w145]
    tunnel: string[] ["time", "temp", "Bx", "By", "Bz", "Vsource", "Lockin0", "Lockin1", "Lockin2", "Lockin3", "Lockin4", "Lockin5", "B_rate", "DC0", "DC1", "DC2", "DC3", "DC4", "DC5", "DC6", "DC7"] ("wavenames (.Vx, etc)") -> [_ w144]
    tunnel: w74 -> [_ w143]
    frame False {
    }
    frame True {
      n77 = call <userlib>:"LV to ITX AutoPlot.vi"("filename"=w145, "path"=w147, "Notes"=w146, "Data"=w143, "wavenames (.Vx, etc)"=w144) -> ()  [unwired: 10 in, 1 out]
    }
  }
  "B fields" <- w26
